vi "new batch buffer.vi"() -> (3 "buffer":refnum<data-value>)   [LabVIEW 2020, in "nominal core steps.lvlib"]
doc: "A buffer allowing TestStand to collect individual points for several channels and stream them all at once, for efficiency. For a simple single-channel buffer, use the point buffer."
uses:
  nominal core steps.lvlib
  channel uid.ctl
  single point.ctl
  points buffer.ctl
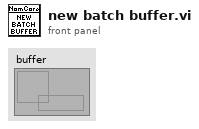
[diagram p1: front panel]
types:
  T1 = typedef "nominal core steps.lvlib/channel uid.ctl" = cluster{"channel name":string, "tags":map{string, string}}
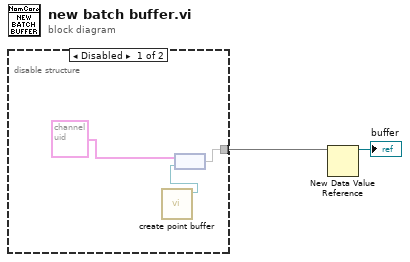
[diagram p0: block diagram]
diagram:
  n1 = disable-structure shown="Disabled" {
    disable-tunnel: [w3 _] -> w2
    frame Disabled {
      n2 = call "create point buffer.vi"() -> ("point buffer"=w4:refnum<data-value>)  [unwired: 10 in, 1 out]
      n3 = node(T1 {"channel name"="", "tags"={}} ("channel unique identifier"), w4) -> (w3:map{T1, refnum<data-value>})
    }
    frame Enabled {
    }
  }
  n4 = New Data Value Reference(data value=w2) -> (data value reference=→"buffer":refnum<data-value>)  [unwired: 1 in, 1 out]
